vi "Test ISO 8601 Round Trip.vi"(8 "error in (no error)":errorcluster, 10 "Work Folder":path, 11 "Test Data Folder":path) -> (0 "error out":errorcluster, 2 "Report":string, 3 "Passed":bool)   [LabVIEW 2024]
doc: "Checks Timestamp to ISO 8601 UTC.vi and ISO 8601 UTC to Timestamp.vi: a timestamp with milliseconds survives the round trip exactly, timestamp 0 and the empty string map onto each other, and a malformed string is error 5001.\n\nInputs: Test Data Folder holds the source copies (Samples, v1); each run works in a new case folder under Work Folder. Passed is TRUE when every check passed and no error occurred; Report lists every check.\n\nGenerated by: Claude"
uses:
  Utilities/Time Management/Time Management.lvlib
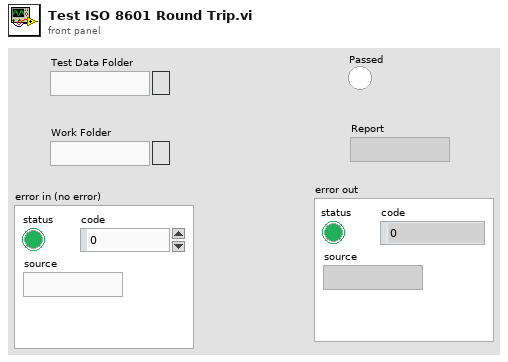
[diagram p1: front panel]
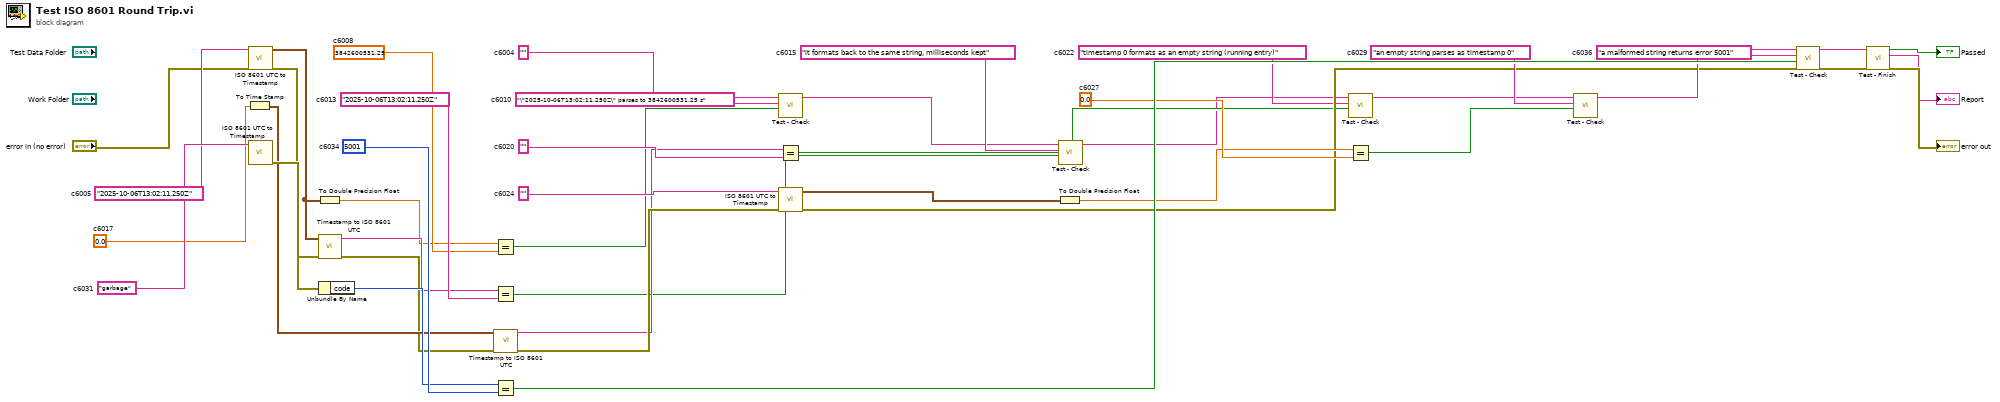
[diagram p0: block diagram]
diagram:
  w38 = "a malformed string returns error 5001"  # c6036
  w36 = 5001  # c6034
  w33 = "garbage"  # c6031
  w31 = "an empty string parses as timestamp 0"  # c6029
  w29 = 0.0  # c6027
  w25 = ""  # c6024
  w23 = "timestamp 0 formats as an empty string (running entry)"  # c6022
  w21 = ""  # c6020
  w17 = 0.0  # c6017
  w15 = "it formats back to the same string, milliseconds kept"  # c6015
  w13 = "2025-10-06T13:02:11.250Z"  # c6013
  w9 = "\"2025-10-06T13:02:11.250Z\" parses to 3842600531.25 s"  # c6010
  w7 = 3842600531.25  # c6008
  w3 = "2025-10-06T13:02:11.250Z"  # c6005
  w2 = ""  # c6004
  n1 = call "ISO 8601 UTC to Timestamp.vi"("error in (no error)"="error in (no error)", "ISO 8601 UTC"=w3) -> ("error out"=w5:errorcluster, "Timestamp"=w4:timestamp)  [unwired: 8 in]
  n2 = To Time Stamp(1:w17) -> (0:w18:timestamp)
  n3 = call "ISO 8601 UTC to Timestamp.vi"("ISO 8601 UTC"=w33) -> ("error out"=w34:errorcluster)  [unwired: 9 in, 1 out]
  n4 = To Double Precision Float(number=w4) -> (double precision float=w6:dbl)
  n5 = call "Timestamp to ISO 8601 UTC.vi"("error in (no error)"=w5, "Timestamp"=w4) -> ("error out"=w12:errorcluster, "ISO 8601 UTC"=w11:string)  [unwired: 8 in]
  n6 = Unbundle By Name(w34) -> ("code"=w35:i32)
  n7 = Equal?(x=w6, y=w7) -> (x = y?=w8:bool)
  n8 = Equal?(x=w11, y=w13) -> (x = y?=w14:bool)
  n9 = call "Timestamp to ISO 8601 UTC.vi"("error in (no error)"=w12, "Timestamp"=w18) -> ("error out"=w20:errorcluster, "ISO 8601 UTC"=w19:string)  [unwired: 8 in]
  n10 = Equal?(x=w35, y=w36) -> (x = y?=w37:bool)
  n11 = call "Test - Check.vi"("Condition"=w8, "Check Name"=w9, "Report in"=w2) -> ("Report out"=w10:string)  [unwired: 7 in, 1 out]
  n12 = Equal?(x=w19, y=w21) -> (x = y?=w22:bool)
  n13 = call "ISO 8601 UTC to Timestamp.vi"("error in (no error)"=w20, "ISO 8601 UTC"=w25) -> ("error out"=w27:errorcluster, "Timestamp"=w26:timestamp)  [unwired: 8 in]
  n14 = call "Test - Check.vi"("Condition"=w14, "Check Name"=w15, "Report in"=w10) -> ("Report out"=w16:string)  [unwired: 7 in, 1 out]
  n15 = To Double Precision Float(number=w26) -> (double precision float=w28:dbl)
  n16 = call "Test - Check.vi"("Condition"=w22, "Check Name"=w23, "Report in"=w16) -> ("Report out"=w24:string)  [unwired: 7 in, 1 out]
  n17 = Equal?(x=w28, y=w29) -> (x = y?=w30:bool)
  n18 = call "Test - Check.vi"("Condition"=w30, "Check Name"=w31, "Report in"=w24) -> ("Report out"=w32:string)  [unwired: 7 in, 1 out]
  n19 = call "Test - Check.vi"("Condition"=w37, "Check Name"=w38, "Report in"=w32) -> ("Report out"=w39:string)  [unwired: 7 in, 1 out]
  n20 = call "Test - Finish.vi"("error in (no error)"=w27, "Report"=w39) -> ("error out"=→"error out":errorcluster, "Report out"=→"Report":string, "Passed"=→"Passed":bool)  [unwired: 7 in]
